vi "Creating_admin_Login.vi"(8 "error in (no error)":errorcluster) -> (0 "error out":errorcluster)   [LabVIEW 2021]
panel:
  in  "Add User":bool
  in  "Password":string
  in  "User Name":string
  # "ADD USER"
  # "Give User Name and Password"
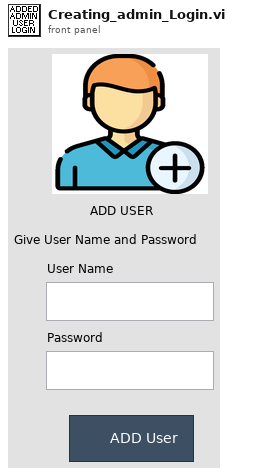
[diagram p1: front panel]
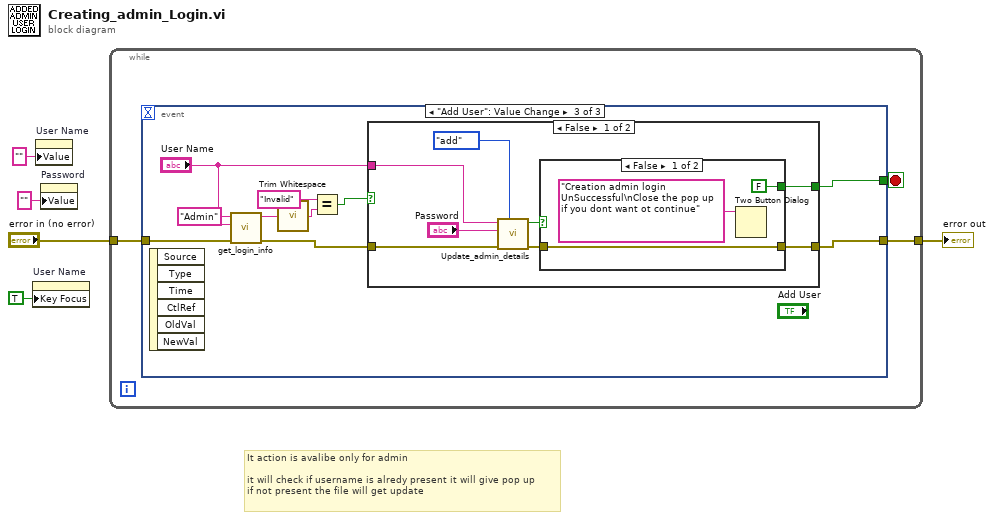
[diagram p0: block diagram]
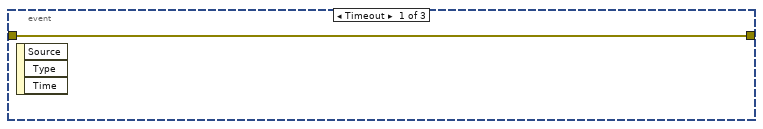
[diagram p2: hidden frame]
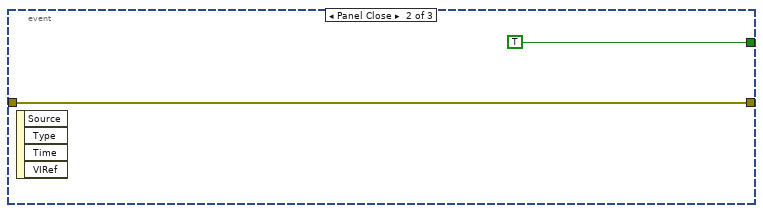
[diagram p3: hidden frame]
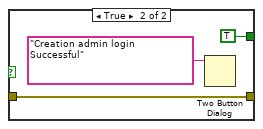
[diagram p4: hidden frame]
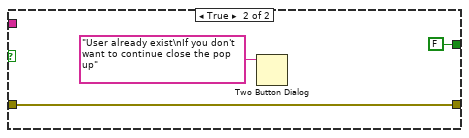
[diagram p5: hidden frame]
diagram:
  # "It action is avalibe only for admin\n\nit will check if username is alredy present it will give pop up\nif not present the file will get update"
  n1 = property on="User Name" class="Str"("Key Focus"=TRUE) -> ()  [unwired: 2 in, 2 out]
  n2 = property on="User Name" class="Str"("Value"="" ("User Name")) -> ()  [unwired: 2 in, 2 out]
  n3 = property on="Password" class="Str"("Value"="" ("Password")) -> ()  [unwired: 2 in, 2 out]
  n4 = while {
    tunnel: "error in (no error)" -> [w7]
    tunnel: [w6] -> w4
    stop <- w8 stop-if-true
    n5 = event shown="[2] \"Add User\": Value Change" {
      selector: _ -> [_ _ _]
      dyn-events: _ -> [_ _ _]
      timeout: _ -> [_ _ _]
      tunnel: [_ TRUE w21] -> w8
      tunnel: w7 -> [w9 w11 w19]
      tunnel: [w9 w11 w20] -> w6
      event Timeout {
        n6 = event-data() -> ()  [unwired: 1 in, 3 out]
      }
      event Panel Close {
        n7 = event-data() -> ()  [unwired: 1 in, 4 out]
      }
      event "Add User": Value Change {
        n8 = event-data() -> ()  [unwired: 1 in, 6 out]
        n9 = call "get_login_info.vi"("error in (no error)"=w19, "User name"="User Name", "User"="Admin") -> ("error out"=w18:errorcluster, "User_name"=w17:string)  [unwired: 6 in, 1 out]
        n10 = call <vilib>:"Trim Whitespace.vi"("string"=w17) -> ("trimmed string"=w14:string)  [unwired: 1 in]
        n11 = Equal?(x="Invalid", y=w14) -> (x = y?=w15:bool)
        n12 = case shown="False" w15 {
          tunnel: [w26 FALSE] -> w21
          tunnel: w18 -> [w25 w36]
          tunnel: [w24 w36] -> w20
          tunnel: "User Name" -> [w22 _]
          frame False {
            n13 = call "Update_admin_details.vi"("Enum"=enum16{"add", "update", "read"}."add", "error in (no error)"=w25, "string"="Password", "User"=w22) -> ("error out"=w23:errorcluster, "Status"=w27:bool)  [unwired: 6 in]
            n14 = case shown="False" w27 {
              tunnel: [FALSE TRUE] -> w26
              tunnel: [w30 w33] -> w24
              tunnel: w23 -> [w30 w33]
              frame False {
                n15 = Two Button Dialog(message="Creation admin login UnSuccessful\nClose the pop up if you dont want ot continue") -> ()  [unwired: 2 in, 1 out]
              }
              frame True {
                n16 = Two Button Dialog(message="Creation admin login Successful") -> ()  [unwired: 2 in, 1 out]
              }
            }
          }
          frame True {
            n17 = Two Button Dialog(message="User already exist\nIf you don't want to continue close the pop up") -> ()  [unwired: 2 in, 1 out]
          }
        }
      }
    }
  }
  "error out" <- w4
